vi "Configuration Files.vi"(8 "error in (no error)":errorcluster, 11 "Node Ptr":T3 format="%.0x") -> (0 "error out":errorcluster)   [LabVIEW 2020, in "AIM ARINC 429 System Explorer.lvlib" / "Implementation.lvlib"]
uses:
  Implementation.lvlib
  <vilib>/NI VeriStand/Custom Device API/Custom Device API.lvlib
  <vilib>/NI VeriStand/Custom Device Tools/Custom Device Utility Library/Custom Device Utility Library.lvlib
  Types/Browse Button.ctl
  Types/Path Control.ctl
  Scripting/AIM/AIM ARINC 429 Scripting.lvlib
  <vilib>/NI VeriStand/Custom Device API/Custom Device Item Ref.ctl
  Types/Configuration Files Page Data.ctl
panel:
  in  "Refresh":bool
  in  "Parameters":T1
  in  "SHDocVw.IWebBrowser":refnum<k7>(container)
  in  "General Header":cluster{"Section Name":string}={"Section Name"="AIM ARINC 429 - Configuration Files"}
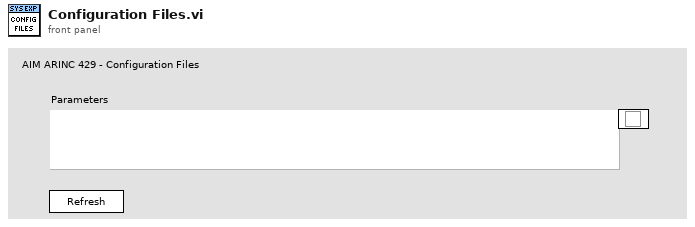
[diagram p1: front panel]
types:
  T1 = typedef "AIM ARINC 429 System Explorer.lvlib/Implementation.lvlib/Path Control.ctl" = cluster{"file path":path, "Browse":T2}
  T2 = typedef "AIM ARINC 429 System Explorer.lvlib/Implementation.lvlib/Browse Button.ctl" = bool
  T3 = typedef "Custom Device API.lvlib/Custom Device Item Ref.ctl" = u64
  T4 = typedef "AIM ARINC 429 System Explorer.lvlib/Implementation.lvlib/Configuration Files Page Data.ctl" = cluster{"Parameters":T1, "most recent parameters path":path, "custom device ref":T3, "MD5":string, "CD scripted?":bool, "parameters path ctl ref":refnum<vi>}
  T5 = typedef "Custom Device API.lvlib/Custom Device Commands.ctl" = enum16{"Default", "Item renamed", "Shutdown", "Dynamic button pressed"}
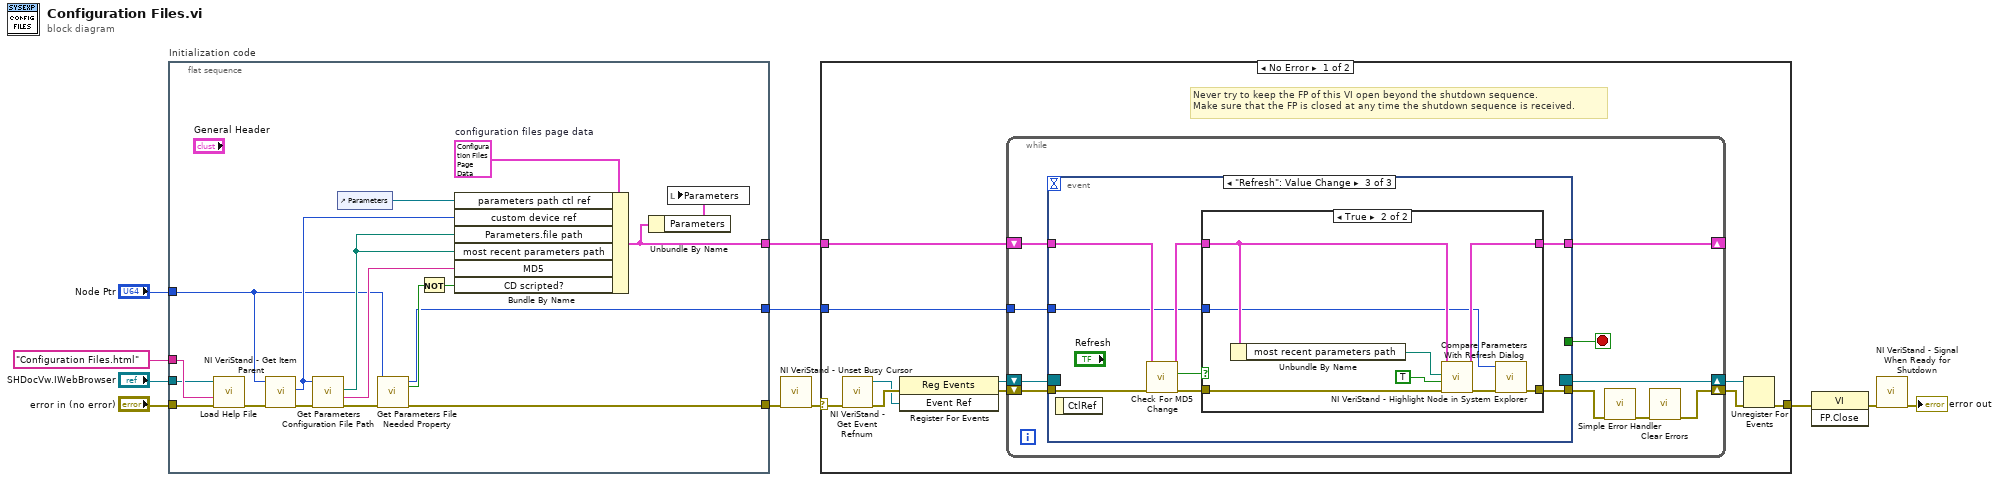
[diagram p0: block diagram]
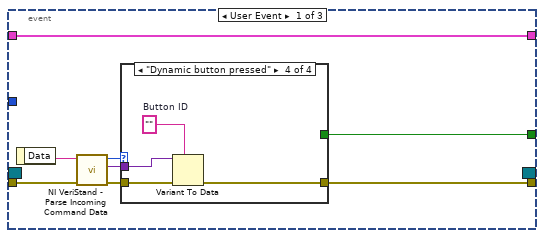
[diagram p2: hidden frame]
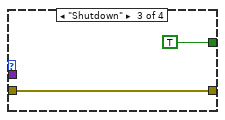
[diagram p5: hidden frame]
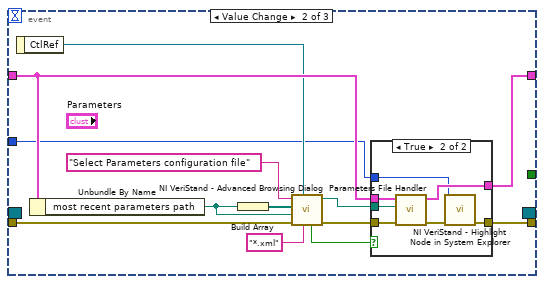
[diagram p6: hidden frame]
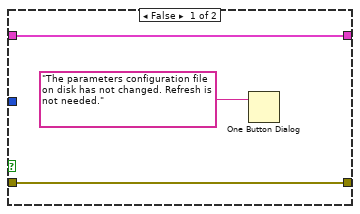
[diagram p8: hidden frame]
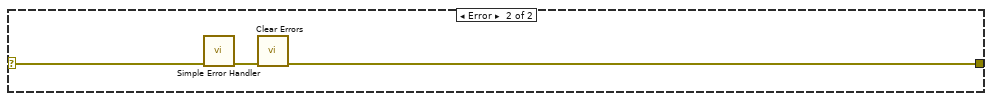
[diagram p9: hidden frame]
diagram:
  n1 = flat-sequence "Initialization code" {
    tunnel: "error in (no error)" -> [w29]
    tunnel: "Node Ptr" -> [w16]
    tunnel: [w17] -> w7
    tunnel: "SHDocVw.IWebBrowser" -> [w23]
    tunnel: "Configuration Files.html" ("CD_CHM_Section") -> [w28]
    tunnel: [w21] -> w2
    tunnel: [w12] -> w1
    frame #0 {
      w27 = T4 {"Parameters"={"file path"=path "", "Browse"=FALSE}, "most recent parameters path"=path "", "custom device ref"=0, "MD5"="", "CD scripted?"=FALSE, "parameters path ctl ref"=refnum}  # configuration files page data
      n2 = call "Load Help File.vi"("error in (no error)"=w29, "HTML File to Load"=w28, "Browser"=w23) -> ("error out"=w25:errorcluster)  [unwired: 8 in]
      n3 = call <vilib>:"NI VeriStand - Get Item Parent.vi"("error in (no error)"=w25, "Item Ref in"=w16) -> ("error out"=w13:errorcluster, "Parent Ref"=w24:T3)  [unwired: 6 in, 2 out]
      n4 = call "Get Parameters Configuration File Path.vi"("error in"=w13, "custom device ref"=w24) -> ("error out"=w18:errorcluster, "MD5 checksum"=w20:string, "parameters configuration file path"=w22:path)  [unwired: 6 in, 1 out]
      n5 = control-ref of="Parameters"() -> (w19:refnum<vi>)
      n6 = call "Get Parameters File Needed Property.vi"("error in"=w18, "configuration files ref"=w16) -> ("error out"=w17:errorcluster, "needed"=w15:bool, "configuration files ref out"=w12:T3)  [unwired: 7 in]
      n7 = Not(x=w15) -> (.not. x?=w14:bool)
      n8 = Bundle By Name(cluster=w27, "parameters path ctl ref"=w19, "custom device ref"=w24, "Parameters.file path"=w22, "most recent parameters path"=w22, "MD5"=w20, "CD scripted?"=w14) -> (w21:T4)
      n9 = Unbundle By Name(w21) -> ("Parameters"=w26:T1)
      n10 = local write "Parameters"(w26) -> ()
    }
  }
  n11 = call <vilib>:"NI VeriStand - Unset Busy Cursor.vi"("error in (no error)"=w7) -> ("error out"=w6:errorcluster)  [unwired: 10 out]
  n12 = case shown="No Error" w6 {
    selector: w6 -> [w32 w109]
    tunnel: [w36 w107] -> w11
    tunnel: w2 -> [w31 _]
    tunnel: w1 -> [w30 _]
    frame No Error {
      # "Never try to keep the FP of this VI open beyond the shutdown sequence.\nMake sure that the FP is closed at any time the shutdown sequence is received."
      n13 = call <vilib>:"NI VeriStand - Get Event Refnum.vi"("error in (no error)"=w32) -> ("error out"=w39:errorcluster, "Event Ref"=w35:refnum<user-event>)  [unwired: 9 out]
      n14 = register-events(error in=w39, w35) -> (reference out=w33:refnum<event-registration>, error out=w34:errorcluster)  [unwired: 1 in]
      n15 = while {
        shift-right: [w43] -> w37
        shift-left: w34 -> [w48]
        shift-right: [w49] -> w38
        shift-left: w33 -> [w47]
        shift-right: [w41] -> _
        shift-left: w31 -> [w42]
        tunnel: w30 -> [w40]
        stop <- w46 stop-if-true
        n16 = event shown="[2] \"Refresh\": Value Change" {
          selector: w47 -> [_ _ _]
          dyn-events: [_ _ _] -> w49
          timeout: _ -> [_ _ _]
          tunnel: w48 -> [w57 w78 w92]
          tunnel: [w53 _ _] -> w46
          tunnel: [w52 w68 w95] -> w45
          tunnel: w42 -> [w50 w72 w89]
          tunnel: [w50 w71 w94] -> w41
          tunnel: w40 -> [_ w66 w88]
          event User Event {
            n17 = event-data() -> ("Data"=w56:string)  [unwired: 1 out]
            n18 = call <vilib>:"NI VeriStand - Parse Incoming Command Data.vi"("error in (no error)"=w57, "Incoming data"=w56) -> ("error out"=w55:errorcluster, "Outgoing data"=w51:variant, "Action"=w54:T5)  [unwired: 7 out]
            n19 = case shown="\"Dynamic button pressed\"" w54 {
              tunnel: w55 -> [w58 w59 w60 w65]
              tunnel: [_ _ TRUE _] -> w53
              tunnel: [w58 w59 w60 w62] -> w52
              tunnel: w51 -> [_ _ _ w64]
              frame "Default", Default {
              }
              frame "Item renamed" {
              }
              frame "Shutdown" {
              }
              frame "Dynamic button pressed" {
                w63 = ""  # Button ID
                n20 = Variant To Data(error in=w65, type=w63, Variant=w64) -> (error out=w62:errorcluster)  [unwired: 1 out]
              }
            }
          }
          event Value Change {
            n21 = event-data() -> ("CtlRef"=w70:refnum<vi>)  [unwired: 1 out]
            n22 = Unbundle By Name(w72) -> ("most recent parameters path"=w74:path)
            n23 = Build Array(w74) -> (w76:path[])
            n24 = call <vilib>:"NI VeriStand - Advanced Browsing Dialog.vi"("File Pattern"="*.xml", "CtlRef"=w70, "error in (no error)"=w78, "Most recent path"=w74, "Paths"=w76, "Dialog Title"="Select Parameters configuration file") -> ("error out"=w73:errorcluster, "Selected file"=w69:path, "Valid?"=w67:bool)  [unwired: 2 in, 1 out]
            n25 = case shown="True" w67 {
              tunnel: w73 -> [w79 w87]
              tunnel: w72 -> [w80 w86]
              tunnel: [w80 w85] -> w71
              tunnel: w69 -> [_ w84]
              tunnel: [w79 w82] -> w68
              tunnel: w66 -> [_ w81]
              frame False {
              }
              frame True {
                n26 = call "Parameters File Handler.vi"("error in"=w87, "selected parameters file"=w84, "configuration files page data in"=w86) -> ("error out"=w83:errorcluster, "configuration files page data out"=w85:T4)  [unwired: 7 in]
                n27 = call <vilib>:"NI VeriStand - Highlight Node in System Explorer.vi"("error in (no error)"=w83, "Item Ref in"=w81) -> ("error out"=w82:errorcluster)  [unwired: 8 in, 1 out]
              }
            }
          }
          event "Refresh": Value Change {
            n28 = event-data() -> ()  [unwired: 2 out]
            n29 = call "Check For MD5 Change.vi"("error in"=w92, "configuration files page data"=w89) -> ("error out"=w91:errorcluster, "MD5 change?"=w90:bool, "configuration files page data out"=w93:T4)  [unwired: 7 in]
            n30 = case shown="True" w90 {
              tunnel: [w97 w100] -> w95
              tunnel: w91 -> [w97 w106]
              tunnel: w93 -> [w96 w105]
              tunnel: [w96 w103] -> w94
              tunnel: w88 -> [_ w99]
              frame False {
                n31 = One Button Dialog(message="The parameters configuration file on disk has not changed. Refresh is not needed.") -> ()  [unwired: 1 in, 1 out]
              }
              frame True {
                n32 = Unbundle By Name(w105) -> ("most recent parameters path"=w104:path)
                n33 = call "Compare Parameters With Refresh Dialog.vi"("error in"=w106, "refresh button"=TRUE, "selected parameters file"=w104, "configuration files page data in"=w105) -> ("error out"=w101:errorcluster, "configuration files page data out"=w103:T4)  [unwired: 6 in]
                n34 = call <vilib>:"NI VeriStand - Highlight Node in System Explorer.vi"("error in (no error)"=w101, "Item Ref in"=w99) -> ("error out"=w100:errorcluster)  [unwired: 8 in, 1 out]
              }
            }
          }
        }
        n35 = call <vilib>:"Simple Error Handler.vi"("error in (no error)"=w45) -> ("error out"=w44:errorcluster)  [unwired: 1 in, 7 out]
        n36 = call <vilib>:"Clear Errors.vi"("error in (no error)"=w44) -> ("error out"=w43:errorcluster)  [unwired: 1 in, 5 out]
      }
      n37 = Unregister For Events(event registration refnum=w38, error in=w37) -> (error out=w36:errorcluster)
    }
    frame Error {
      n38 = call <vilib>:"Simple Error Handler.vi"("error in (no error)"=w109) -> ("error out"=w108:errorcluster)  [unwired: 1 in, 7 out]
      n39 = call <vilib>:"Clear Errors.vi"("error in (no error)"=w108) -> ("error out"=w107:errorcluster)  [unwired: 1 in, 5 out]
    }
  }
  n40 = invoke class="VI" method="FP.Close"(error in=w11) -> (error out=w10:errorcluster)  [unwired: 2 in, 2 out]
  n41 = call <vilib>:"NI VeriStand - Signal When Ready for Shutdown.vi"("error in (no error)"=w10) -> ("error out"=→"error out":errorcluster)  [unwired: 10 out]
